vi "csb encode can to ws.vi"(0 "id":u32, 1 "data":u8[](array[numeric]), 2 "mask":u32, 3 "out_cap":i32, 5 "ide":u8, 7 "fdf":u8, 9 "brs":u8, 11 "error in (no error)":errorcluster, 12 "len":i32, 13 "out":u8[](array[numeric])) -> (4 "out out":u8[](array[numeric]), 6 "function return":i32, 15 "error out":errorcluster)   [LabVIEW 2021, in "CANsub_Codec.lvlib"]
doc: "int32_t csb_encode_can_to_ws(uint32_t id, uint8_t ide, uint8_t fdf, uint8_t brs,\n const uint8_t *data, int32_t len, uint32_t mask,\n uint8_t *out, int32_t out_cap);"
uses:
  CANsub_Codec.lvlib
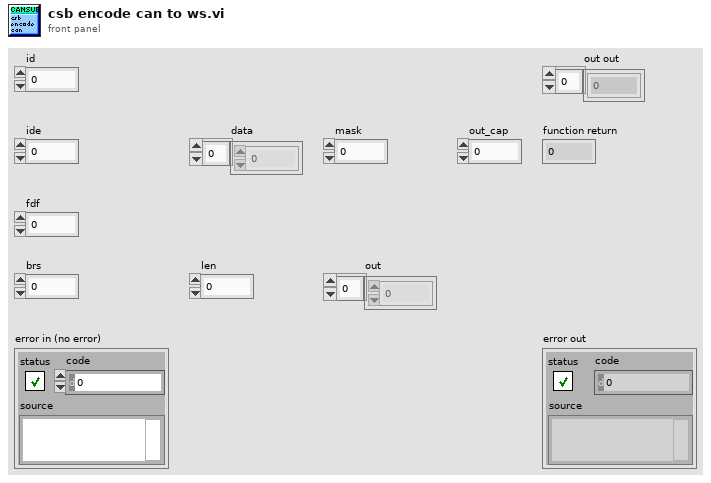
[diagram p1: front panel]
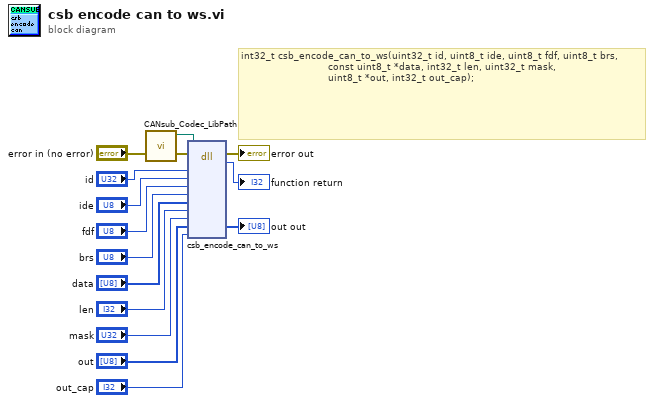
[diagram p0: block diagram]
diagram:
  # "int32_t csb_encode_can_to_ws(uint32_t id, uint8_t ide, uint8_t fdf, uint8_t brs,\n                             const uint8_t *data, int32_t len, uint32_t mask,\n                             uint8_t *out, int32_t out_cap);"
  n1 = call "CANsub_Codec_LibPath.vi"() -> ("Path"=w1:path)  [unwired: 11 in]
  n2 = dll-call lib="libcansub_codec.*" fn="csb_encode_can_to_ws"(path in=w1, error in="error in (no error)", "id"="id", "ide"="ide", "fdf"="fdf", "brs"="brs", "data"="data", "len"="len", "mask"="mask", "out"="out", "out_cap"="out_cap") -> (error out=→"error out":errorcluster, "return type"=→"function return":i32, "out"=→"out out":u8[])  [unwired: 9 in, 1 out]
